vi "Handle Error.vi"(8 "error in (no error)":errorcluster, 11 "Measurement in":refnum<class "Measurement.lvclass">) -> (0 "error out":errorcluster, 2 "stop actor?":bool=TRUE, 3 "Measurement out":refnum<class "Measurement.lvclass">)   [LabVIEW 2017, in "Measurement Actor.lvlib" / "Measurement.lvclass"]
doc: "(<B>Filename</B>: Actor Framework.lvlib:Actor.lvclass:Handle Error.vi)\n\nDefines how the actor handles an error that occurred while processing a message.\n\nBy default, this method does nothing except stop the actor. This method also treats error code 43 (coming from <B>error in</B>) as a sign that the actor shut down normally. In this situation, the Handle Error method does not return the error on <B>error out</B>, meaning the actor's caller will not receive it. All other error codes will be returned on <B>error out</B>.\n\nA descendant class may override this method to change this behavior."
uses:
  Measurement.lvclass
  C:/Program Files (x86)/National Instruments/LabVIEW 2017/vi.lib/ActorFramework/Actor/Actor.lvclass
  <vilib>/ActorFramework/Actor/Actor.lvclass/Actor.ctl
  <vilib>/ActorFramework/Message Enqueuer/Message Enqueuer.lvclass/Message Enqueuer.ctl
  <vilib>/ActorFramework/Message Enqueuer/Init from Existing Queue.vi
  <vilib>/ActorFramework/Message Enqueuer/Enqueue.vi
  Messages/Close Msg/Close Msg.lvclass
  C:/Program Files (x86)/National Instruments/LabVIEW 2017/vi.lib/ActorFramework/Message/Message.lvclass
  <vilib>/ActorFramework/Message Priority Queue/Priority Enqueue.vi
  <vilib>/ActorFramework/Actor/Actor.lvclass
  <vilib>/ActorFramework/Message Enqueuer/Message Enqueuer.lvclass
  Controller/Messages/Log Status/Log Status.lvclass
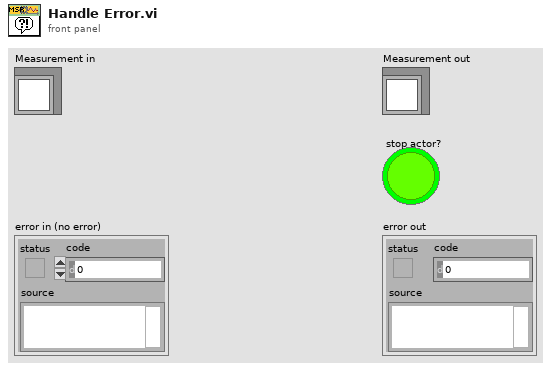
[diagram p1: front panel]
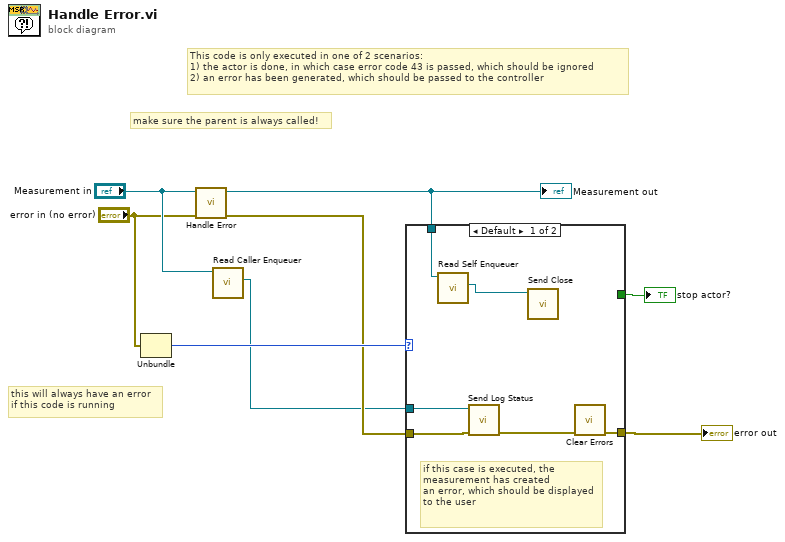
[diagram p0: block diagram]
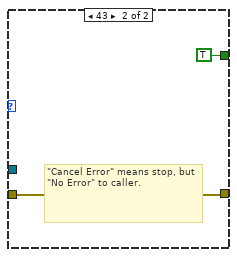
[diagram p2: hidden frame]
diagram:
  # "make sure the parent is always called!"
  # "this will always have an error\nif this code is running"
  # "This code is only executed in one of 2 scenarios:\n1) the actor is done, in which case error code 43 is passed, which should be ignored\n2) an error has been generated, which should be passed to the controller"
  n1 = Unbundle("error in (no error)") -> ("code"=w8:i32)  [unwired: 2 out]
  n2 = call-parent "Handle Error.vi"("error in (no error)"="error in (no error)", "Actor in"="Measurement in") -> ("error out"=w4:errorcluster, "Actor out"=w5:refnum<class "Measurement.lvclass">)  [unwired: 7 in, 1 out]
  "Measurement out" <- w5
  n3 = call <vilib>:"Read Caller Enqueuer.vi"("Actor"="Measurement in") -> ("Caller Enqueuer"=w1:refnum<class "Message Enqueuer.lvclass">)  [unwired: 10 in]
  n4 = case shown="Default" w8 {
    tunnel: [_ TRUE ("stop actor?")] -> w7
    tunnel: w5 -> [w14 _]
    tunnel: w4 -> [w10 w15]
    tunnel: [w12 w15] -> w3
    tunnel: w1 -> [w11 _]
    frame Default {
      # "if this case is executed, the measurement has created\nan error, which should be displayed to the user"
      n5 = call <vilib>:"Read Self Enqueuer.vi"("Actor"=w14) -> ("Self Enqueuer"=w13:refnum<class "Message Enqueuer.lvclass">)  [unwired: 10 in]
      n6 = call "Send Log Status.vi"("error in (no error)"=w10, "Message Enqueuer in"=w11) -> ("error out"=w9:errorcluster)  [unwired: 8 in, 1 out]
      n7 = call "Send Close.vi"("Message Enqueuer in"=w13) -> ()  [unwired: 9 in, 2 out]
      n8 = call <vilib>:"Clear Errors.vi"("error in (no error)"=w9) -> ("error out"=w12:errorcluster)  [unwired: 5 in, 1 out]
    }
    frame 43 {
      # "\"Cancel Error\" means stop, but \"No Error\" to caller."
    }
  }
  "error out" <- w3
  "stop actor?" <- w7
